vi "Envoi mail.vi"(2 "Objet":string="test", 3 "Message":string="envoi liste mail", 5 "Mail liste":string[](array[string])=["christine.nicolas@ias.u-psud.fr"]) -> ()   [LabVIEW 2022 SP3]
uses:
  Variables globales/Variable glob mails.vi
  Variables globales/Variable glob generale.vi
  Mails/Copie de NI_SMTPEmail.lvlib
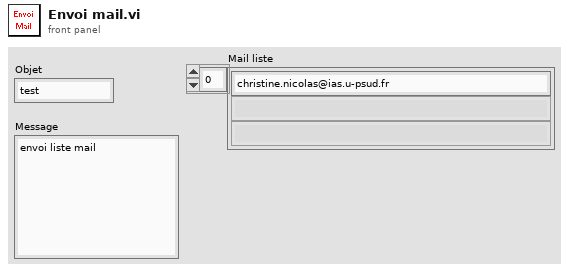
[diagram p1: front panel]
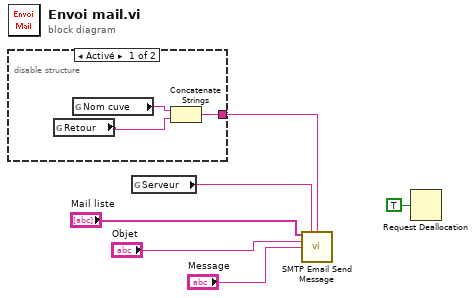
[diagram p0: block diagram]
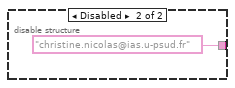
[diagram p2: hidden frame]
diagram:
  n1 = disable-structure shown="Activé" {
    disable-tunnel: [w8 "christine.nicolas@ias.u-psud.fr"] -> w5
    frame Enabled {
      n2 = global read "Variable glob mails.vi" "Retour"() -> (w7:string)
      n3 = global read "Variable glob generale.vi" "Nom cuve"() -> (w9:string)
      n4 = Concatenate Strings(w9, w7) -> (w8:string)
    }
    frame Disabled {
    }
  }
  n5 = global read "Variable glob mails.vi" "Serveur"() -> (w1:string)
  n6 = call "SMTP Email Send Message.vi"("recipients"="Mail liste", "mail server"=w1, "return address"=w5, "subject ([No Subject])"="Objet", "message"="Message") -> ()  [unwired: 9 in, 2 out]
  n7 = Request Deallocation(TRUE ("flag")) -> ()
